vi "Display Loader.vi"(8 "error in (no error)":errorcluster, 11 "VI in":refnum<vi>) -> (0 "error out":errorcluster)   [LabVIEW 2019, in "gRPC Template Creation Utility.lvlib"]
uses:
  gRPC Template Creation Utility.lvlib
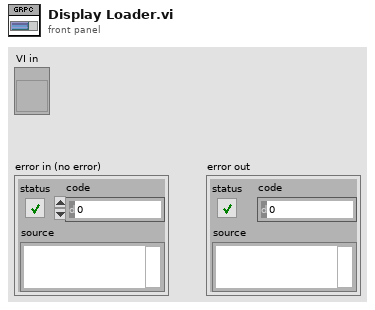
[diagram p1: front panel]
types:
  T1 = enum16{"Always On", "Always Off", "Off While Running"}
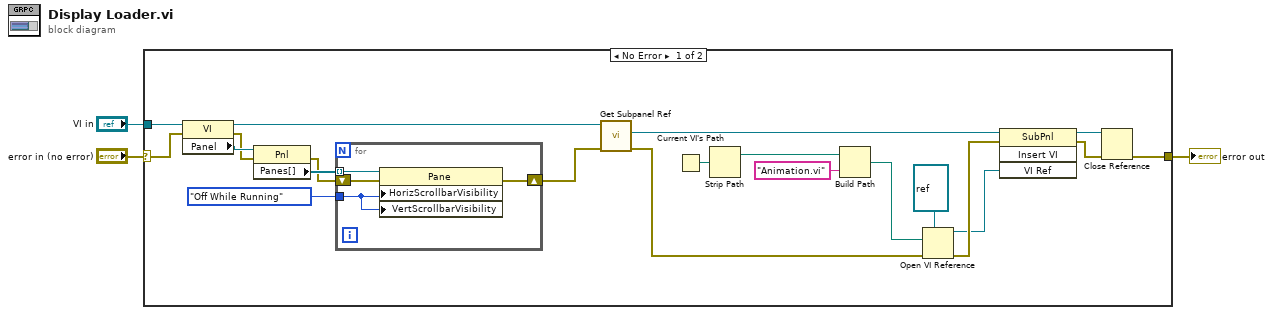
[diagram p0: block diagram]
diagram:
  n1 = case shown="No Error" "error in (no error)" {
    selector: "error in (no error)" -> [w5 w29]
    tunnel: [w13 w29] -> w3
    tunnel: "VI in" -> [w12 _]
    frame No Error {
      n2 = property class="VI"(reference=w12, error in=w5) -> (reference out=w8:refnum<vi>, error out=w7:errorcluster, "Panel"=w11:refnum<vi>)
      n3 = property class="Pnl"(reference=w11, error in=w7) -> (error out=w6:errorcluster, "Panes[]"=w10:refnum<vi>[])  [unwired: 1 out]
      n4 = for {
        tunnel: w10 -> [w28] mode=indexing
        tunnel: T1."Off While Running" ("Horizontal Scrollbar Visibility") -> [w27]
        shift-right: [w25] -> w4
        shift-left: w6 -> [w26]
        n5 = property class="Pane"(reference=w28, error in=w26, "HorizScrollbarVisibility"=w27, "VertScrollbarVisibility"=w27) -> (error out=w25:errorcluster)  [unwired: 1 out]
      }
      n6 = call "Get Subpanel Ref.vi"("error in (no error)"=w4, "Owner VI in"=w8) -> ("error out"=w16:errorcluster, "SubPanel out"=w24:refnum<vi>)  [unwired: 8 in]
      n7 = Current VI's Path() -> (path=w21:path)
      n8 = Strip Path(path=w21) -> (stripped path=w22:path)  [unwired: 1 out]
      n9 = Build Path(base path=w22, name or relative path="Animation.vi") -> (appended path=w15:path)
      n10 = Open VI Reference(type specifier VI Refnum (for type only)=refnum<vi> refnum, vi path=w15, error in (no error)=w16) -> (vi reference=w14:refnum<vi>, error out=w20:errorcluster)  [unwired: 3 in]
      n11 = invoke class="SubPnl" method="Insert VI"(reference=w24, error in=w20, "VI Ref"=w14) -> (reference out=w18:refnum<vi>, error out=w19:errorcluster)  [unwired: 1 in, 2 out]
      n12 = Close Reference(reference=w18, error in (no error)=w19) -> (error out=w13:errorcluster)
    }
    frame Error {
    }
  }
  "error out" <- w3
